vi "俄罗斯方块.vi"() -> ()   [LabVIEW 2021]
uses:
  <vilib>/Utility/config.llb/Read Key (U32).vi
  <vilib>/Utility/config.llb/Read Key (Boolean).vi
  <vilib>/Utility/config.llb/Read Key (I32).vi
  <vilib>/Utility/config.llb/Write Key (U32).vi
  <vilib>/Utility/config.llb/Write Key (Boolean).vi
  <vilib>/Utility/config.llb/Write Key (I32).vi
  <vilib>/Utility/config.llb/NI_LVConfig.lvlib
panel:
  out "扫描代码":i16
  out "键按下状态":bool=TRUE
  out "初始化状态":bool=TRUE
  out "配置文件路径":path
  out "结束状态":bool=TRUE
  out "落下状态":bool=TRUE
  in  "下落触发源":bool=TRUE
  out "速度":i32
  in  "开始/暂停":bool
  out "最多行数":u32
  out "最高分数":u32
  out "行数":u32
  out "分数":u32
  in  "退出":bool
  out "当前形状数组":u32[][](array[colorbox])
  out "Y":i8
  out "X":i8
  out "颜色盒":u32(colorbox)
  in  "新形状触发源":bool=TRUE
  in  "绘图触发源":bool=TRUE
  out "新形状数组":u32[][](array[colorbox])
  out "主窗数组":u32[][](array[colorbox])
  out "二维图片":picture
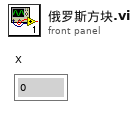
[diagram p1: front panel]
types:
  T1 = typedef "NI_LVConfig.lvlib/Config Data RefNum.ctl" = refnum<k1>
  T2 = enum16{"Left Button", "Center Button", "Right Button", "Window Close"}
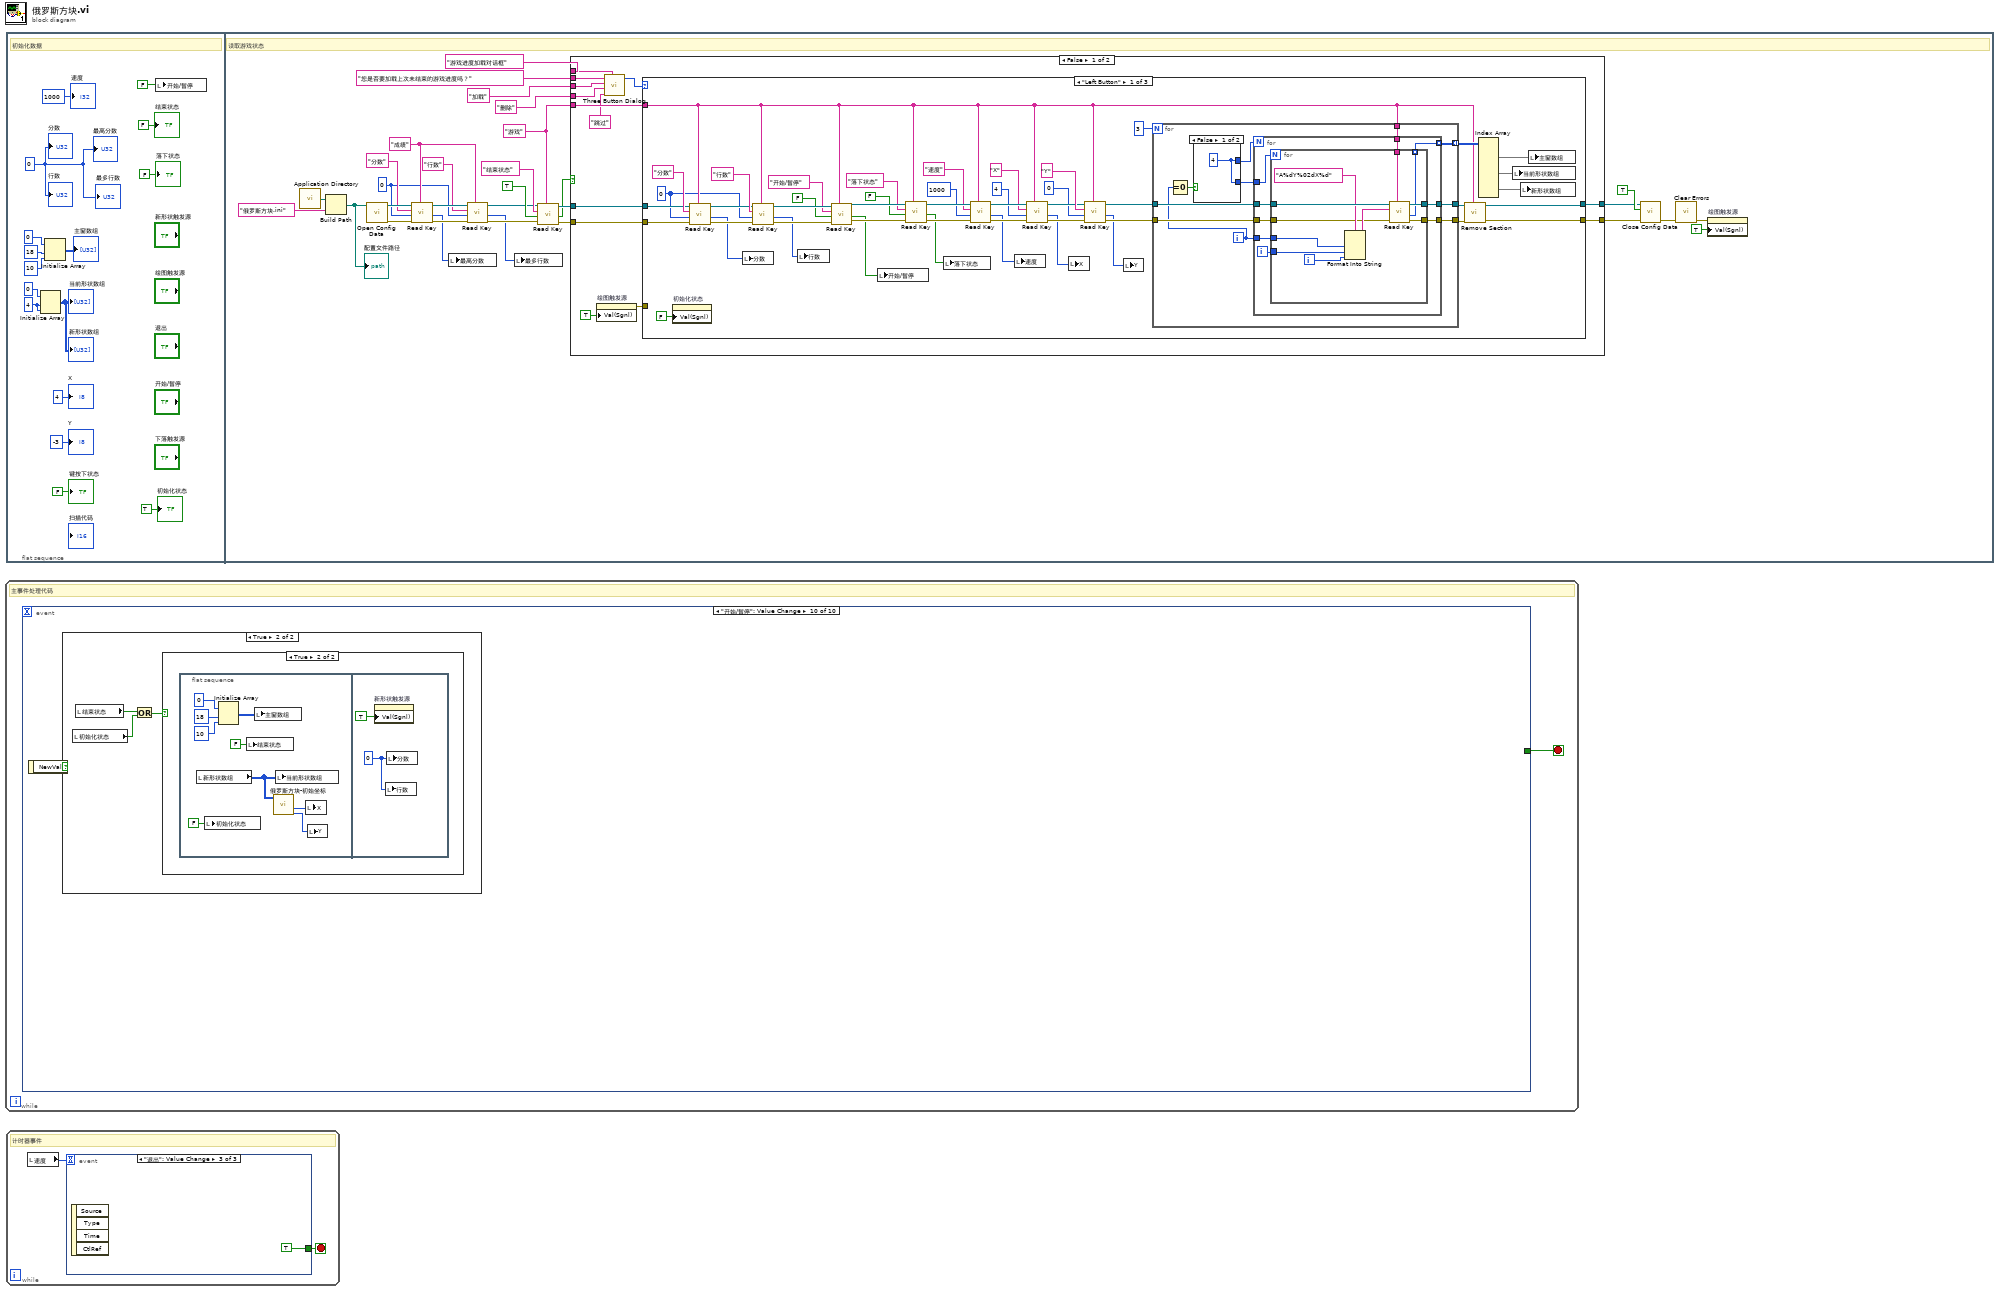
[diagram p0: block diagram]
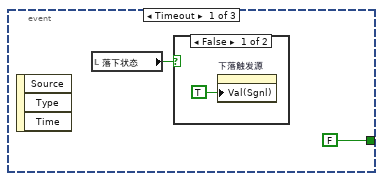
[diagram p2: hidden frame]
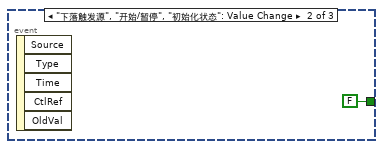
[diagram p4: hidden frame]
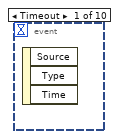
[diagram p5: hidden frame]
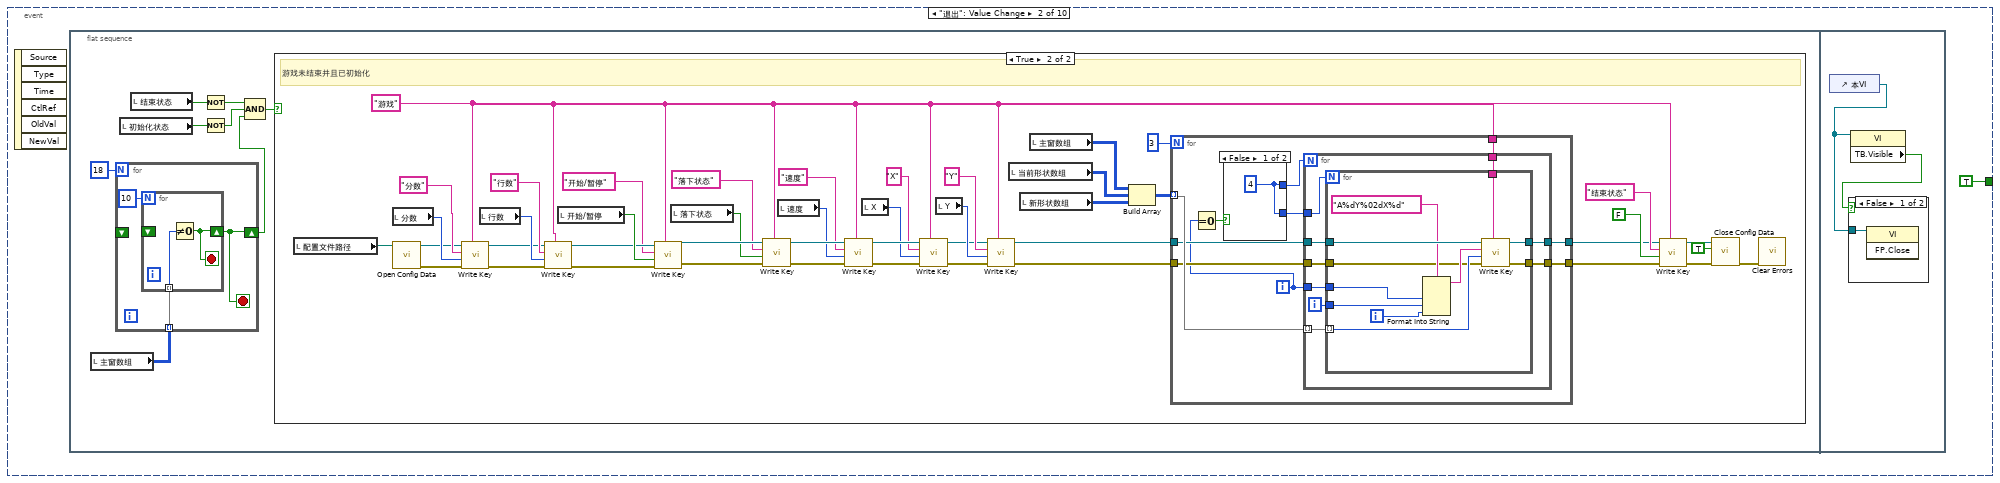
[diagram p6: hidden frame]
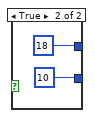
[diagram p8: hidden frame]
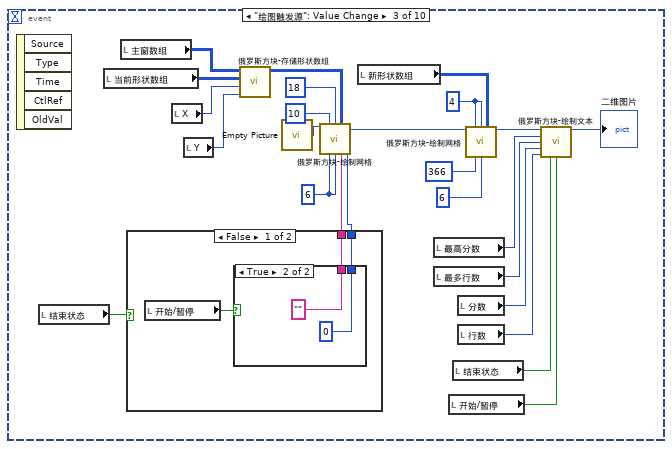
[diagram p10: hidden frame]
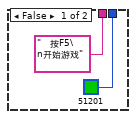
[diagram p11: hidden frame]
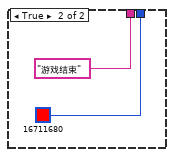
[diagram p12: hidden frame]
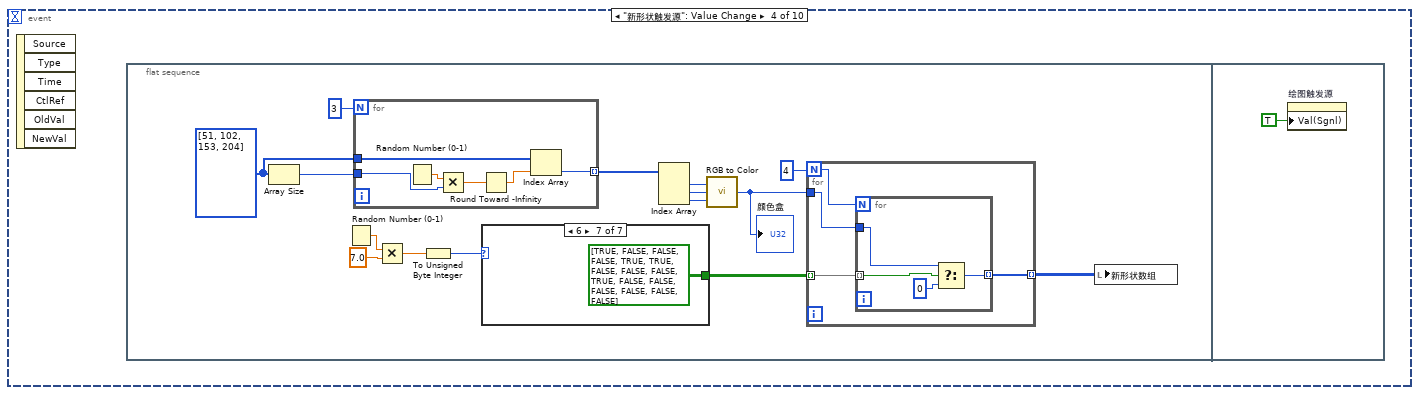
[diagram p13: hidden frame]
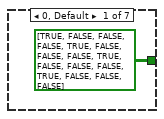
[diagram p14: hidden frame]
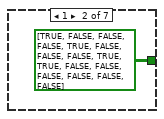
[diagram p15: hidden frame]
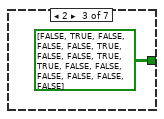
[diagram p16: hidden frame]
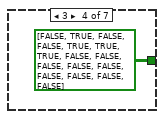
[diagram p17: hidden frame]
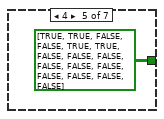
[diagram p18: hidden frame]
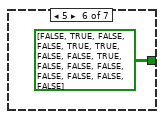
[diagram p19: hidden frame]
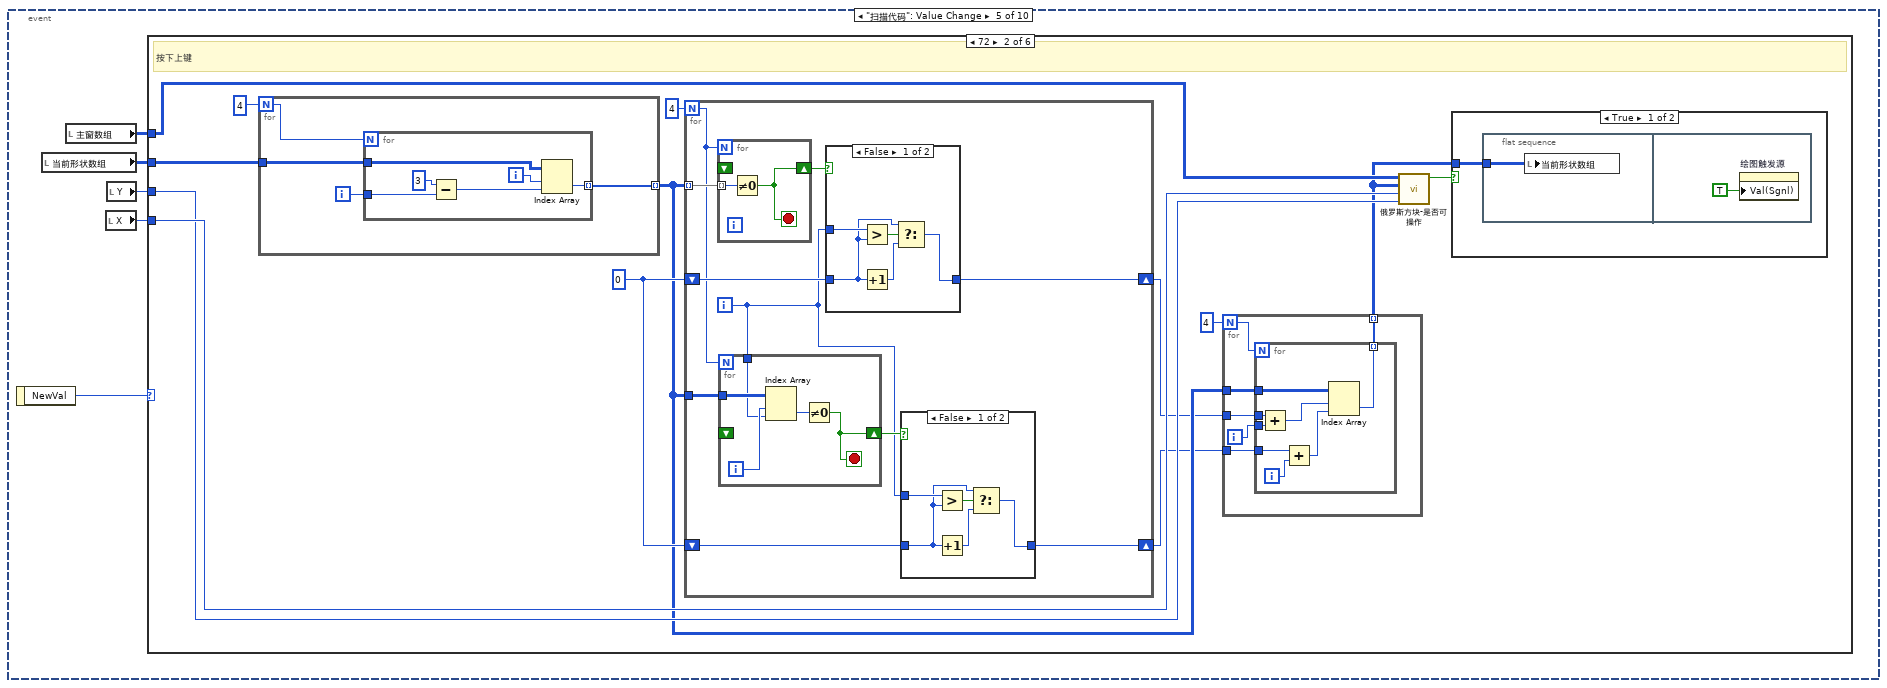
[diagram p20: hidden frame]
diagram:
  n1 = while {
    stop <- w1 stop-if-true
    # "主事件处理代码"
    n2 = event shown="[9] \"开始/暂停\": Value Change" {
      selector: _ -> [_ _ _ _ _ _ _ _ _ _]
      dyn-events: _ -> [_ _ _ _ _ _ _ _ _ _]
      timeout: _ -> [_ _ _ _ _ _ _ _ _ _]
      tunnel: [_ TRUE _ _ _ _ _ _ _ _] -> w1
      event Timeout {
        n3 = event-data() -> ()  [unwired: 1 in, 3 out]
      }
      event "退出": Value Change {
        n4 = event-data() -> ()  [unwired: 1 in, 6 out]
        n5 = flat-sequence {
          frame #0 {
            n6 = local read "主窗数组"() -> (w4:u32[][])
            n7 = for {
              N: 18 -> [_]
              shift-right: [w11] -> w3
              shift-left: _ -> [_]
              tunnel: w4 -> [w12] mode=indexing
              stop <- w11 stop-if-true
              n8 = for {
                N: 10 -> [_]
                shift-right: [w14] -> w11
                shift-left: _ -> [_]
                tunnel: w12 -> [w15] mode=indexing
                stop <- w14 stop-if-true
                n9 = Not Equal To 0?(x=w15) -> (x != 0?=w14:bool)
              }
            }
            n10 = local read "初始化状态"() -> (w7:bool)
            n11 = local read "结束状态"() -> (w8:bool)
            n12 = Not(x=w8) -> (.not. x?=w9:bool)
            n13 = Not(x=w7) -> (.not. x?=w6:bool)
            n14 = Compound Arithmetic op=AND ("复合运算")(w9, w6, w3) -> (w10:bool)
            n15 = case shown="True" w10 {
              frame False {
                # "不保存状态"
              }
              frame True {
                w16 = "游戏" ("section")
                # "游戏未结束并且已初始化"
                n16 = local read "配置文件路径"() -> (w60:path)
                n17 = local read "分数"() -> (w57:u32)
                n18 = call <vilib>:"Open Config Data.vi"("configuration file path"=w60) -> ("error out"=w46:errorcluster, "refnum"=w47:T1)  [unwired: 8 in, 1 out]
                n19 = call-poly <vilib>:"Write Key.vi"("section"=w16, "error in (no error)"=w46, "value"=w57, "key"="分数", "refnum"=w47) -> ("error out"=w53:errorcluster, "refnum out"=w54:T1)  [unwired: 4 in, 1 out]
                n20 = local read "行数"() -> (w56:u32)
                n21 = call-poly <vilib>:"Write Key.vi"("section"=w16, "error in (no error)"=w53, "value"=w56, "key"="行数", "refnum"=w54) -> ("error out"=w44:errorcluster, "refnum out"=w43:T1)  [unwired: 4 in, 1 out]
                n22 = local read "开始/暂停"() -> (w45:bool)
                n23 = call-poly <vilib>:"Write Key.vi"("section"=w16, "error in (no error)"=w44, "value"=w45, "key"="开始/暂停", "refnum"=w43) -> ("error out"=w40:errorcluster, "refnum out"=w41:T1)  [unwired: 4 in, 1 out]
                n24 = local read "落下状态"() -> (w39:bool)
                n25 = call-poly <vilib>:"Write Key.vi"("section"=w16, "error in (no error)"=w40, "value"=w39, "key"="落下状态", "refnum"=w41) -> ("error out"=w36:errorcluster, "refnum out"=w37:T1)  [unwired: 4 in, 1 out]
                n26 = local read "速度"() -> (w34:i32)
                n27 = call-poly <vilib>:"Write Key.vi"("section"=w16, "error in (no error)"=w36, "value"=w34, "key"="速度", "refnum"=w37) -> ("error out"=w33:errorcluster, "refnum out"=w32:T1)  [unwired: 4 in, 1 out]
                n28 = local read "X"() -> (w30:i8)
                n29 = call-poly <vilib>:"Write Key.vi"("section"=w16, "error in (no error)"=w33, "value"=w30, "key"="X", "refnum"=w32) -> ("error out"=w29:errorcluster, "refnum out"=w26:T1)  [unwired: 4 in, 1 out]
                n30 = local read "Y"() -> (w28:i8)
                n31 = call-poly <vilib>:"Write Key.vi"("section"=w16, "error in (no error)"=w29, "value"=w28, "key"="Y", "refnum"=w26) -> ("error out"=w19:errorcluster, "refnum out"=w20:T1)  [unwired: 4 in, 1 out]
                n32 = local read "当前形状数组"() -> (w24:u32[][])
                n33 = local read "新形状数组"() -> (w25:u32[][])
                n34 = local read "主窗数组"() -> (w23:u32[][])
                n35 = Build Array(w23, w24, w25) -> (w22:u32[][][])
                n36 = for {
                  N: 3 -> [_]
                  tunnel: w22 -> [w70] mode=indexing
                  tunnel: w20 -> [w69]
                  tunnel: w19 -> [w68]
                  tunnel: [w67] -> w18
                  tunnel: [w66] -> w17
                  tunnel: w16 -> [w65]
                  i -> [w64]
                  n37 = Equal To 0?(x=w64) -> (x = 0?=w63:bool)
                  n38 = case shown="False" w63 {
                    tunnel: [w71 18] -> w62
                    tunnel: [w71 10] -> w61
                    frame False {
                      w71 = 4
                    }
                    frame True {
                    }
                  }
                  n39 = for {
                    N: w62 -> [_]
                    tunnel: w61 -> [w82]
                    tunnel: w70 -> [w81] mode=indexing
                    tunnel: w69 -> [w80]
                    tunnel: w64 -> [w78]
                    tunnel: w68 -> [w77]
                    tunnel: [w76] -> w67
                    tunnel: [w75] -> w66
                    tunnel: w65 -> [w74]
                    i -> [w79]
                    n40 = for {
                      N: w82 -> [_]
                      tunnel: w81 -> [w87] mode=indexing
                      tunnel: w80 -> [w93]
                      tunnel: w79 -> [w91]
                      tunnel: w78 -> [w90]
                      tunnel: w77 -> [w86]
                      tunnel: [w85] -> w76
                      tunnel: [w84] -> w75
                      tunnel: w74 -> [w83]
                      i -> [w89]
                      n41 = Format Into String(format string="A%dY%02dX%d" ("格式字符串"), w90, w91, w89) -> (resulting string=w92:string)  [unwired: 2 in, 1 out]
                      n42 = call-poly <vilib>:"Write Key.vi"("section"=w83, "error in (no error)"=w86, "value"=w87, "key"=w92, "refnum"=w93) -> ("error out"=w84:errorcluster, "refnum out"=w85:T1)  [unwired: 4 in, 1 out]
                    }
                  }
                }
                n43 = call-poly <vilib>:"Write Key.vi"("section"=w16, "error in (no error)"=w17, "value"=FALSE, "key"="结束状态", "refnum"=w18) -> ("error out"=w52:errorcluster, "refnum out"=w51:T1)  [unwired: 4 in, 1 out]
                n44 = call <vilib>:"Close Config Data.vi"("error in (no error)"=w52, "write file if changed (T)"=TRUE, "refnum"=w51) -> ("error out"=w59:errorcluster)  [unwired: 7 in, 1 out]
                n45 = call <vilib>:"Clear Errors.vi"("error in (no error)"=w59) -> ()  [unwired: 5 in, 2 out]
              }
            }
          }
          frame #1 {
            n46 = control-ref of="本VI"() -> (w95:refnum<vi>)
            n47 = property class="VI"(reference=w95) -> ("TB.Visible"=w94:bool)  [unwired: 1 in, 2 out]
            n48 = case shown="False" w94 {
              tunnel: w95 -> [w96 _]
              frame False {
                n49 = invoke class="VI" method="FP.Close"(reference=w96) -> ()  [unwired: 2 in, 3 out]
              }
              frame True {
              }
            }
          }
        }
      }
      event "绘图触发源": Value Change {
        w114 = i16 4 ("yN")
        w108 = i16 6 ("xOffset")
        n50 = event-data() -> ()  [unwired: 1 in, 5 out]
        n51 = local read "结束状态"() -> (w111:bool)
        n52 = local read "当前形状数组"() -> (w97:u32[][])
        n53 = local read "主窗数组"() -> (w98:u32[][])
        n54 = case shown="False" w111 {
          tunnel: [w124 "游戏结束"] -> w110
          tunnel: [w123 u32 16711680 ("消息颜色")] -> w109
          frame False {
            n55 = local read "开始/暂停"() -> (w122:bool)
            n56 = case shown="True" w122 {
              tunnel: ["　按F5\n开始游戏" ""] -> w124
              tunnel: [u32 51201 ("消息颜色") u32 0 ("消息颜色")] -> w123
              frame False {
              }
              frame True {
              }
            }
          }
          frame True {
          }
        }
        n57 = local read "X"() -> (w117:i8)
        n58 = local read "Y"() -> (w116:i8)
        n59 = call "俄罗斯方块-存储形状数组.vi"("Y"=w116, "X"=w117, "当前形状数组"=w97, "主窗数组输入"=w98) -> ("主窗数组输出"=w99:u32[][])  [unwired: 4 in, 1 out]
        n60 = call "Empty Picture"() -> ("empty picture"=w120:picture)
        n61 = call "俄罗斯方块-绘制网格.vi"("图片输入"=w120, "xN"=i16 10, "yN"=i16 18, "数组"=w99, "xOffset"=w108, "yOffset"=w108, "消息文本"=w110, "消息颜色"=w109) -> ("图片输出"=w121:picture)  [unwired: 7 in]
        n62 = local read "新形状数组"() -> (w113:u32[][])
        n63 = local read "最高分数"() -> (w102:u32)
        n64 = local read "最多行数"() -> (w103:u32)
        n65 = local read "开始/暂停"() -> (w100:bool)
        n66 = local read "结束状态"() -> (w101:bool)
        n67 = local read "分数"() -> (w104:u32)
        n68 = local read "行数"() -> (w105:u32)
        n69 = call "俄罗斯方块-绘制网格.vi"("图片输入"=w121, "xN"=w114, "yN"=w114, "数组"=w113, "xOffset"=i16 366, "yOffset"=i16 6) -> ("图片输出"=w107:picture)  [unwired: 9 in]
        n70 = call "俄罗斯方块-绘制文本.vi"("输入图片"=w107, "最高分数"=w102, "最多行数"=w103, "分数"=w104, "行数"=w105, "结束状态"=w101, "开始/暂停"=w100) -> ("输出图片"=→"二维图片":picture)  [unwired: 8 in]
      }
      event "新形状触发源": Value Change {
        n71 = event-data() -> ()  [unwired: 1 in, 6 out]
        n72 = flat-sequence {
          frame #0 {
            w133 = u8[] [51, 102, 153, 204]
            n73 = Array Size(array=w133) -> (size(s)=w134:i32)
            n74 = Random Number (0-1)() -> (number: 0 to 1=w139:dbl)
            n75 = for {
              N: 3 -> [_]
              tunnel: [w163] -> w144 mode=indexing
              tunnel: w134 -> [w165]
              tunnel: w133 -> [w164]
              n76 = Random Number (0-1)() -> (number: 0 to 1=w166:dbl)
              n77 = Multiply(x=w166, y=w165) -> (x*y=w161:dbl)
              n78 = Round Toward -Infinity(1:w161) -> (0:w162:dbl)
              n79 = Index Array(array=w164, index=w162) -> (element=w163:u8)
            }
            n80 = Multiply(x=w139, y=7.0) -> (x*y=w138:dbl)
            n81 = To Unsigned Byte Integer(number=w138) -> (unsigned 8bit integer=w140:u8)
            n82 = case shown="6" w140 {
              tunnel: [bool[][] [[TRUE, FALSE, FALSE, FALSE], [TRUE, FALSE, FALSE, FALSE], [TRUE, FALSE, FALSE, FALSE], [TRUE, FALSE, FALSE, FALSE]] bool[][] [[TRUE, FALSE, FALSE, FALSE], [TRUE, FALSE, FALSE, FALSE], [TRUE, TRUE, FALSE, FALSE], [FALSE, FALSE, FALSE, FALSE]] bool[][] [[FALSE, TRUE, FALSE, FALSE], [FALSE, TRUE, FALSE, FALSE], [TRUE, TRUE, FALSE, FALSE], [FALSE, FALSE, FALSE, FALSE]] bool[][] [[FALSE, TRUE, FALSE, FALSE], [TRUE, TRUE, TRUE, FALSE], [FALSE, FALSE, FALSE, FALSE], [FALSE, FALSE, FALSE, FALSE]] bool[][] [[TRUE, TRUE, FALSE, FALSE], [TRUE, TRUE, FALSE, FALSE], [FALSE, FALSE, FALSE, FALSE], [FALSE, FALSE, FALSE, FALSE]] bool[][] [[FALSE, TRUE, FALSE, FALSE], [TRUE, TRUE, FALSE, FALSE], [TRUE, FALSE, FALSE, FALSE], [FALSE, FALSE, FALSE, FALSE]] bool[][] [[TRUE, FALSE, FALSE, FALSE], [TRUE, TRUE, FALSE, FALSE], [FALSE, TRUE, FALSE, FALSE], [FALSE, FALSE, FALSE, FALSE]]] -> w135
              frame 0, Default {
              }
              frame 1 {
              }
              frame 2 {
              }
              frame 3 {
              }
              frame 4 {
              }
              frame 5 {
              }
              frame 6 {
              }
            }
            n83 = Index Array(array=w144) -> (element #1=w143:u8, element #2=w142:u8, element #3=w141:u8)  [unwired: 3 in]
            n84 = call <vilib>:"RGB to Color.vi"("B"=w141, "G"=w142, "R"=w143) -> ("Color"=w132:u32)
            "颜色盒" <- w132
            n85 = for {
              N: 4 -> [w146]
              tunnel: w132 -> [w149]
              tunnel: w135 -> [w148] mode=indexing
              tunnel: [w147] -> w131 mode=indexing
              n86 = for {
                N: w146 -> [_]
                tunnel: w149 -> [w153]
                tunnel: w148 -> [w151] mode=indexing
                tunnel: [w150] -> w147 mode=indexing
                n87 = Select(t=w153, s=w151, f=u32 0) -> (s? t:f=w150:u32)
              }
            }
            n88 = local write "新形状数组"(w131) -> ()
          }
          frame #1 {
            n89 = property on="绘图触发源" class="Bool (strict)"("Val(Sgnl)"=TRUE ("绘图触发源")) -> ()  [unwired: 2 in, 2 out]
          }
        }
      }
      event "扫描代码": Value Change {
        n90 = event-data() -> ("NewVal"=w172:i16)  [unwired: 1 in]
        n91 = local read "当前形状数组"() -> (w170:u32[][])
        n92 = local read "主窗数组"() -> (w171:u32[][])
        n93 = local read "X"() -> (w169:i8)
        n94 = local read "Y"() -> (w168:i8)
        n95 = case shown="72" w172 {
          tunnel: w171 -> [_ w185 _ _ w249 w258]
          tunnel: w170 -> [_ w180 _ _ w248 w257]
          tunnel: w169 -> [_ w184 _ _ w246 w255]
          tunnel: w168 -> [_ w183 _ _ w247 w256]
          frame 0, Default {
          }
          frame 72 {
            w178 = 0
            # "按下上键"
            n96 = for {
              N: 4 -> [w231]
              tunnel: [w232] -> w177 mode=indexing
              tunnel: w180 -> [w230]
              i -> [w229]
              n97 = for {
                N: w231 -> [_]
                tunnel: [w238] -> w232 mode=indexing
                tunnel: w230 -> [w237]
                tunnel: w229 -> [w233]
                i -> [w234]
                n98 = Subtract(x=i8 3, y=w233) -> (x-y=w235:i32)
                n99 = Index Array(array=w237, index (row)=w234, index (col)=w235) -> (element=w238:u32)
              }
            }
            n100 = for {
              N: 4 -> [w205]
              tunnel: w177 -> [w209] mode=indexing
              shift-right: [w206] -> w175
              shift-left: w178 -> [w207]
              tunnel: w177 -> [w204]
              shift-right: [w202] -> w174
              shift-left: w178 -> [w201]
              i -> [w200]
              n101 = for {
                N: w205 -> [_]
                tunnel: w209 -> [w228] mode=indexing
                shift-right: [w227] -> w208
                shift-left: _ -> [_]
                stop <- w227 stop-if-true
                n102 = Not Equal To 0?(x=w228) -> (x != 0?=w227:bool)
              }
              n103 = for {
                N: w205 -> [_]
                tunnel: w204 -> [w220]
                tunnel: w200 -> [w218]
                shift-right: [w216] -> w203
                shift-left: _ -> [_]
                i -> [w219]
                stop <- w216 stop-if-true
                n104 = Index Array(array=w220, index (row)=w219, index (col)=w218) -> (element=w217:u32)
                n105 = Not Equal To 0?(x=w217) -> (x != 0?=w216:bool)
              }
              n106 = case shown="False" w208 {
                tunnel: w207 -> [w223 w226]
                tunnel: [w221 w226] -> w206
                tunnel: w200 -> [w224 _]
                frame False {
                  n107 = Greater?(x=w224, y=w223) -> (0:w225:bool)
                  n108 = Increment(x=w223) -> (x+1=w222:i32)
                  n109 = Select(t=w223, s=w225, f=w222) -> (s? t:f=w221:i32)
                }
                frame True {
                }
              }
              n110 = case shown="False" w203 {
                tunnel: w201 -> [w212 w215]
                tunnel: [w210 w215] -> w202
                tunnel: w200 -> [w213 _]
                frame False {
                  n111 = Greater?(x=w213, y=w212) -> (0:w214:bool)
                  n112 = Increment(x=w212) -> (x+1=w211:i32)
                  n113 = Select(t=w212, s=w214, f=w211) -> (s? t:f=w210:i32)
                }
                frame True {
                }
              }
            }
            n114 = for {
              N: 4 -> [w190]
              tunnel: w177 -> [w191]
              tunnel: w175 -> [w188]
              tunnel: w174 -> [w187]
              tunnel: [w186] -> w173 mode=indexing
              i -> [w189]
              n115 = for {
                N: w190 -> [_]
                tunnel: w191 -> [w199]
                tunnel: w189 -> [w197]
                tunnel: w188 -> [w196]
                tunnel: w187 -> [w194]
                tunnel: [w192] -> w186 mode=indexing
                i -> [w195]
                n116 = Add(x=w196, y=w197) -> (x+y=w198:i32)
                n117 = Add(x=w194, y=w195) -> (x+y=w193:i32)
                n118 = Index Array(array=w199, index (row)=w198, index (col)=w193) -> (element=w192:u32)
              }
            }
            n119 = call "俄罗斯方块-是否可操作.vi"("Y"=w183, "X"=w184, "形状数组"=w173, "主窗数组"=w185) -> ("是否可操作"=w182:bool)  [unwired: 7 in]
            n120 = case shown="True" w182 {
              tunnel: w173 -> [w239 _]
              frame True {
                n121 = flat-sequence {
                  tunnel: w239 -> [w240]
                  frame #0 {
                    n122 = local write "当前形状数组"(w240) -> ()
                  }
                  frame #1 {
                    n123 = property on="绘图触发源" class="Bool (strict)"("Val(Sgnl)"=TRUE ("值(信号)")) -> ()  [unwired: 2 in, 2 out]
                  }
                }
              }
              frame False {
              }
            }
          }
          frame 57 {
            # "空格键"
            n124 = flat-sequence {
              frame #0 {
                n125 = local write "落下状态"(TRUE ("落下状态")) -> ()
              }
              frame #1 {
                n126 = property on="下落触发源" class="Bool (strict)"("Val(Sgnl)"=TRUE ("值(信号)")) -> ()  [unwired: 2 in, 2 out]
              }
            }
          }
          frame 80 {
            # "按下下键"
            n127 = property on="下落触发源" class="Bool (strict)"("Val(Sgnl)"=TRUE ("值(信号)")) -> ()  [unwired: 2 in, 2 out]
          }
          frame 75 {
            # "按下左键"
            n128 = Decrement(x=w246) -> (x-1=w245:i8)
            n129 = call "俄罗斯方块-是否可操作.vi"("Y"=w247, "X"=w245, "形状数组"=w248, "主窗数组"=w249) -> ("是否可操作"=w250:bool)  [unwired: 7 in]
            n130 = case shown="True" w250 {
              tunnel: w245 -> [_ w251]
              frame False {
              }
              frame True {
                n131 = flat-sequence {
                  tunnel: w251 -> [w252]
                  frame #0 {
                    n132 = local write "X"(w252) -> ()
                  }
                  frame #1 {
                    n133 = property on="绘图触发源" class="Bool (strict)"("Val(Sgnl)"=TRUE ("值(信号)")) -> ()  [unwired: 2 in, 2 out]
                  }
                }
              }
            }
          }
          frame 77 {
            # "按下右键"
            n134 = Increment(x=w255) -> (x+1=w254:i8)
            n135 = call "俄罗斯方块-是否可操作.vi"("Y"=w256, "X"=w254, "形状数组"=w257, "主窗数组"=w258) -> ("是否可操作"=w259:bool)  [unwired: 7 in]
            n136 = case shown="True" w259 {
              tunnel: w254 -> [_ w260]
              frame False {
              }
              frame True {
                n137 = flat-sequence {
                  tunnel: w260 -> [w261]
                  frame #0 {
                    n138 = local write "X"(w261) -> ()
                  }
                  frame #1 {
                    n139 = property on="绘图触发源" class="Bool (strict)"("Val(Sgnl)"=TRUE ("值(信号)")) -> ()  [unwired: 2 in, 2 out]
                  }
                }
              }
            }
          }
        }
      }
      event Key Down {
        n140 = event-data() -> ("ScanCode"=w263:i16)  [unwired: 1 in]
        n141 = case shown="63" w263 {
          selector: w263 -> [w264 _ _]
          frame 0, Default {
            n142 = local read "开始/暂停"() -> (w268:bool)
            n143 = local read "落下状态"() -> (w266:bool)
            n144 = Not(x=w266) -> (.not. x?=w267:bool)
            n145 = And(x=w268, y=w267) -> (x .and. y?=w265:bool)
            n146 = case shown="True" w265 {
              tunnel: w264 -> [_ w269]
              frame False {
              }
              frame True {
                n147 = property on="扫描代码" class="DigNum (strict)"("Val(Sgnl)"=w269) -> ()  [unwired: 2 in, 2 out]
              }
            }
            n148 = local write "键按下状态"(w265) -> ()
          }
          frame 63 {
            # "按下F5键"
            n149 = local read "开始/暂停"() -> (w270:bool)
            n150 = Not(x=w270) -> (.not. x?=w271:bool)
            n151 = property on="开始/暂停" class="Bool (strict)"("Val(Sgnl)"=w271) -> ()  [unwired: 2 in, 2 out]
          }
          frame 62 {
            # "按下F4键"
            n152 = property on="退出" class="Bool (strict)"("Val(Sgnl)"=TRUE ("值(信号)")) -> ()  [unwired: 2 in, 2 out]
          }
        }
      }
      event event type 5.0.x8000000b {
        n153 = event-data() -> ("ScanCode"=w275:i16)  [unwired: 1 in]
        n154 = local read "落下状态"() -> (w277:bool)
        n155 = local read "键按下状态"() -> (w276:bool)
        n156 = local read "开始/暂停"() -> (w279:bool)
        n157 = Not(x=w277) -> (.not. x?=w278:bool)
        n158 = Compound Arithmetic op=AND ("复合运算")(w279, w278, w276) -> (w274:bool)
        n159 = case shown="True" w274 {
          tunnel: w275 -> [_ w280]
          frame False {
          }
          frame True {
            n160 = property on="扫描代码" class="DigNum (strict)"("Val(Sgnl)"=w280) -> ()  [unwired: 2 in, 2 out]
          }
        }
        n161 = Not(x=w274) -> (.not. x?=w273:bool)
        n162 = event-data("Discard?"=w273) -> ()  [unwired: 1 in, 1 out]
      }
      event Key Up {
        n163 = event-data() -> ()  [unwired: 1 in, 1 out]
        n164 = local write "键按下状态"(FALSE ("键按下状态")) -> ()
      }
      event "下落触发源": Value Change {
        n165 = event-data() -> ()  [unwired: 1 in, 3 out]
        n166 = local read "开始/暂停"() -> (w282:bool)
        n167 = case shown="True" w282 {
          frame False {
          }
          frame True {
            n168 = local read "当前形状数组"() -> (w287:u32[][])
            n169 = local read "主窗数组"() -> (w288:u32[][])
            n170 = local read "Y"() -> (w285:i8)
            n171 = local read "X"() -> (w286:i8)
            n172 = Increment(x=w285) -> (x+1=w283:i8)
            n173 = call "俄罗斯方块-是否可操作.vi"("Y"=w283, "X"=w286, "形状数组"=w287, "主窗数组"=w288) -> ("是否可操作"=w284:bool)  [unwired: 7 in]
            n174 = case shown="True" w284 {
              tunnel: w283 -> [_ w359]
              tunnel: w285 -> [w289 _]
              frame False {
                # "不可下落，存储，如果结束把结束状态设置为F，否则创建新形状并重新下落"
                n175 = stacked-sequence {
                  tunnel: w289 -> [w296 _ _]
                  frame #0 {
                    # "存储并消除满行和记分"
                    n176 = local read "当前形状数组"() -> (w299:u32[][])
                    n177 = local read "主窗数组"() -> (w298:u32[][])
                    n178 = local read "X"() -> (w297:i8)
                    n179 = call "俄罗斯方块-存储形状数组.vi"("Y"=w296, "X"=w297, "当前形状数组"=w299, "主窗数组输入"=w298) -> ("是否溢出"=w290:bool, "主窗数组输出"=w295:u32[][])  [unwired: 4 in]
                    n180 = local write "结束状态"(w290) -> ()
                    n181 = call "俄罗斯方块-消除满行.vi"("输入数组"=w295) -> ("行数"=w291:u32, "分数"=w292:u32, "输出数组"=w294:u32[][])  [unwired: 8 in]
                    n182 = Greater Than 0?(x=w291) -> (x > 0?=w293:bool)
                    n183 = local write "主窗数组"(w294) -> ()
                    n184 = case shown="True" w293 {
                      tunnel: w292 -> [_ w314]
                      tunnel: w291 -> [_ w315]
                      frame False {
                      }
                      frame True {
                        w308 = 50.0 ("y")
                        n185 = local read "分数"() -> (w305:u32)
                        n186 = local read "行数"() -> (w304:u32)
                        n187 = local read "最多行数"() -> (w302:u32)
                        n188 = local read "最高分数"() -> (w303:u32)
                        n189 = Add(x=w314, y=w305) -> (x+y=w301:u32)
                        n190 = Add(x=w304, y=w315) -> (x+y=w300:u32)
                        n191 = Subtract(x=1000.0, y=w300) -> (x-y=w306:dbl)
                        n192 = Greater?(x=w306, y=w308) -> (0:w310:bool)
                        n193 = Greater?(x=w301, y=w303) -> (0:w312:bool)
                        n194 = Select(t=w306, s=w310, f=w308) -> (s? t:f=w307:dbl)
                        n195 = Greater?(x=w300, y=w302) -> (0:w311:bool)
                        n196 = local write "行数"(w300) -> ()
                        n197 = local write "速度"(w307) -> ()
                        n198 = Or(x=w312, y=w311) -> (x .or. y?=w313:bool)
                        n199 = case shown="True" w313 {
                          tunnel: w312 -> [_ w338]
                          tunnel: w301 -> [_ w337]
                          tunnel: w303 -> [_ w336]
                          tunnel: w311 -> [_ w335]
                          tunnel: w300 -> [_ w334]
                          tunnel: w302 -> [_ w333]
                          frame False {
                          }
                          frame True {
                            w326 = "成绩" ("section")
                            n200 = Select(t=w337, s=w338, f=w336) -> (s? t:f=w317:u32)
                            n201 = Select(t=w334, s=w335, f=w333) -> (s? t:f=w316:u32)
                            n202 = local read "配置文件路径"() -> (w332:path)
                            n203 = local write "最多行数"(w316) -> ()
                            n204 = local write "最高分数"(w317) -> ()
                            n205 = call <vilib>:"Open Config Data.vi"("configuration file path"=w332) -> ("error out"=w327:errorcluster, "refnum"=w328:T1)  [unwired: 8 in, 1 out]
                            n206 = call-poly <vilib>:"Write Key.vi"("section"=w326, "error in (no error)"=w327, "value"=w316, "key"="行数", "refnum"=w328) -> ("error out"=w329:errorcluster, "refnum out"=w330:T1)  [unwired: 4 in, 1 out]
                            n207 = call-poly <vilib>:"Write Key.vi"("section"=w326, "error in (no error)"=w329, "value"=w317, "key"="分数", "refnum"=w330) -> ("error out"=w321:errorcluster, "refnum out"=w322:T1)  [unwired: 4 in, 1 out]
                            n208 = call <vilib>:"Remove Section.vi"("section"="游戏", "error in (no error)"=w321, "refnum"=w322) -> ("error out"=w318:errorcluster, "refnum out"=w319:T1)  [unwired: 6 in, 1 out]
                            n209 = call <vilib>:"Close Config Data.vi"("error in (no error)"=w318, "write file if changed (T)"=TRUE, "refnum"=w319) -> ("error out"=w331:errorcluster)  [unwired: 7 in, 1 out]
                            n210 = call <vilib>:"Clear Errors.vi"("error in (no error)"=w331) -> ()  [unwired: 5 in, 2 out]
                          }
                        }
                        n211 = local write "分数"(w301) -> ()
                      }
                    }
                  }
                  frame #1 {
                    # "初始化落下状态、XY坐标、把新形状作为当前形状"
                    n212 = local read "结束状态"() -> (w339:bool)
                    n213 = local write "落下状态"(FALSE ("落下状态")) -> ()
                    n214 = case shown="False" w339 {
                      frame False {
                        n215 = local read "新形状数组"() -> (w343:u32[][])
                        n216 = call "俄罗斯方块-初始坐标.vi"("输入形状数组"=w343) -> ("Y"=w341:i8, "X"=w342:i8)  [unwired: 9 in]
                        n217 = local write "当前形状数组"(w343) -> ()
                        n218 = local write "X"(w342) -> ()
                        n219 = local write "Y"(w341) -> ()
                      }
                      frame True {
                      }
                    }
                  }
                  frame #2 {
                    # "判断游戏是否结束"
                    n220 = local read "当前形状数组"() -> (w350:u32[][])
                    n221 = local read "主窗数组"() -> (w351:u32[][])
                    n222 = local read "X"() -> (w349:i8)
                    n223 = local read "Y"() -> (w348:i8)
                    n224 = call "俄罗斯方块-是否可操作.vi"("Y"=w348, "X"=w349, "形状数组"=w350, "主窗数组"=w351) -> ("是否可操作"=w345:bool)  [unwired: 7 in]
                    n225 = local read "结束状态"() -> (w347:bool)
                    n226 = Not(x=w347) -> (.not. x?=w346:bool)
                    n227 = And(x=w345, y=w346) -> (x .and. y?=w344:bool)
                    n228 = case shown="False" w344 {
                      frame False {
                        # "游戏结束"
                        n229 = flat-sequence {
                          frame #0 {
                            w355 = 4 ("维数大小")
                            n230 = Initialize Array(u32 0 ("元素"), w355, w355) -> (w353:u32[][])
                            n231 = local write "开始/暂停"(FALSE ("开始/暂停")) -> ()
                            n232 = local write "结束状态"(TRUE ("结束状态")) -> ()
                            n233 = local write "当前形状数组"(w353) -> ()
                          }
                          frame #1 {
                            n234 = property on="绘图触发源" class="Bool (strict)"("Val(Sgnl)"=TRUE ("值(信号)")) -> ()  [unwired: 2 in, 2 out]
                          }
                        }
                      }
                      frame True {
                        # "未结束，产生新形状数据"
                        n235 = property on="新形状触发源" class="Bool (strict)"("Val(Sgnl)"=TRUE ("值(信号)")) -> ()  [unwired: 2 in, 2 out]
                      }
                    }
                  }
                }
              }
              frame True {
                n236 = flat-sequence {
                  tunnel: w359 -> [w360]
                  frame #0 {
                    n237 = local write "Y"(w360) -> ()
                  }
                  frame #1 {
                    n238 = local read "落下状态"() -> (w361:bool)
                    n239 = case shown="False" w361 {
                      frame False {
                        n240 = property on="绘图触发源" class="Bool (strict)"("Val(Sgnl)"=FALSE ("值(信号)")) -> ()  [unwired: 2 in, 2 out]
                      }
                      frame True {
                        n241 = property on="下落触发源" class="Bool (strict)"("Val(Sgnl)"=TRUE ("值(信号)")) -> ()  [unwired: 2 in, 2 out]
                      }
                    }
                  }
                }
              }
            }
          }
        }
      }
      event "开始/暂停": Value Change {
        n242 = event-data() -> ("NewVal"=w364:bool)  [unwired: 1 in]
        n243 = case shown="True" w364 {
          frame False {
            n244 = property on="绘图触发源" class="Bool (strict)"("Val(Sgnl)"=FALSE ("值(信号)")) -> ()  [unwired: 2 in, 2 out]
          }
          frame True {
            n245 = local read "初始化状态"() -> (w367:bool)
            n246 = local read "结束状态"() -> (w368:bool)
            n247 = Or(x=w368, y=w367) -> (x .or. y?=w366:bool)
            n248 = case shown="True" w366 {
              frame False {
                n249 = local read "落下状态"() -> (w369:bool)
                n250 = case shown="True" w369 {
                  frame False {
                    n251 = property on="绘图触发源" class="Bool (strict)"("Val(Sgnl)"=FALSE ("值(信号)")) -> ()  [unwired: 2 in, 2 out]
                  }
                  frame True {
                    n252 = property on="下落触发源" class="Bool (strict)"("Val(Sgnl)"=TRUE ("值(信号)")) -> ()  [unwired: 2 in, 2 out]
                  }
                }
              }
              frame True {
                n253 = flat-sequence {
                  frame #0 {
                    n254 = local read "新形状数组"() -> (w375:u32[][])
                    n255 = local write "初始化状态"(FALSE ("初始化状态")) -> ()
                    n256 = Initialize Array(u32 0 ("元素"), 18 ("维数大小"), 10 ("维数大小")) -> (w377:u32[][])
                    n257 = local write "结束状态"(FALSE ("结束状态")) -> ()
                    n258 = local write "主窗数组"(w377) -> ()
                    n259 = call "俄罗斯方块-初始坐标.vi"("输入形状数组"=w375) -> ("Y"=w373:i8, "X"=w374:i8)  [unwired: 9 in]
                    n260 = local write "当前形状数组"(w375) -> ()
                    n261 = local write "X"(w374) -> ()
                    n262 = local write "Y"(w373) -> ()
                  }
                  frame #1 {
                    w381 = u32 0 ("分数")
                    n263 = property on="新形状触发源" class="Bool (strict)"("Val(Sgnl)"=TRUE ("值(信号)")) -> ()  [unwired: 2 in, 2 out]
                    n264 = local write "行数"(w381) -> ()
                    n265 = local write "分数"(w381) -> ()
                  }
                }
              }
            }
          }
        }
      }
    }
  }
  n266 = while {
    stop <- w383 stop-if-true
    # "计时器事件"
    n267 = local read "速度"() -> (w384:i32)
    n268 = event shown="[2] \"退出\": Value Change" {
      selector: _ -> [_ _ _]
      dyn-events: _ -> [_ _ _]
      timeout: w384 -> [_ _ _]
      tunnel: [FALSE FALSE TRUE] -> w383
      event Timeout {
        n269 = event-data() -> ()  [unwired: 1 in, 3 out]
        n270 = local read "落下状态"() -> (w386:bool)
        n271 = case shown="False" w386 {
          frame False {
            n272 = property on="下落触发源" class="Bool (strict)"("Val(Sgnl)"=TRUE ("值(信号)")) -> ()  [unwired: 2 in, 2 out]
          }
          frame True {
          }
        }
      }
      event "下落触发源", "开始/暂停", "初始化状态": Value Change {
        n273 = event-data() -> ()  [unwired: 1 in, 5 out]
      }
      event "退出": Value Change {
        n274 = event-data() -> ()  [unwired: 1 in, 4 out]
      }
    }
  }
  n275 = flat-sequence {
    frame #0 {
      w390 = u32 0 ("行数")
      w401 = 4 ("维数大小")
      # "初始化数据"
      n276 = Initialize Array(u32 0 ("元素"), w401, w401) -> (→"新形状数组" →"当前形状数组":u32[][])
      n277 = Initialize Array(u32 0 ("元素"), 18 ("维数大小"), 10 ("维数大小")) -> (→"主窗数组":u32[][])
      n278 = local write "开始/暂停"(FALSE ("运行状态")) -> ()
      "分数" <- w390
      "行数" <- w390
      "速度" <- 1000 ("速度")
      "落下状态" <- FALSE ("落下状态")
      "结束状态" <- FALSE ("结束状态")
      "Y" <- i8 -3 ("Y")
      "X" <- i8 4 ("X")
      "初始化状态" <- TRUE ("初始化状态")
      "键按下状态" <- FALSE ("键按下状态")
      "最高分数" <- w390
      "最多行数" <- w390
    }
    frame #1 {
      w422 = "游戏" ("section")
      w428 = "成绩" ("section")
      w408 = u32 0 ("default value")
      # "读取游戏状态"
      n279 = call <vilib>:"Application Directory.vi"() -> ("Application Directory"=w427:path)
      n280 = Build Path(base path=w427, name or relative path="俄罗斯方块.ini" ("名称或相对路径")) -> (appended path=w429:path)
      "配置文件路径" <- w429
      n281 = call <vilib>:"Open Config Data.vi"("configuration file path"=w429) -> ("error out"=w431:errorcluster, "refnum"=w436:T1)  [unwired: 8 in, 1 out]
      n282 = call-poly <vilib>:"Read Key.vi"("section"=w428, "error in (no error)"=w431, "default value"=w408, "key"="分数", "refnum"=w436) -> ("error out"=w432:errorcluster, "value"=w407:u32, "refnum out"=w434:T1)  [unwired: 3 in, 1 out]
      n283 = local write "最高分数"(w407) -> ()
      n284 = call-poly <vilib>:"Read Key.vi"("section"=w428, "error in (no error)"=w432, "default value"=w408, "key"="行数", "refnum"=w434) -> ("error out"=w423:errorcluster, "value"=w406:u32, "refnum out"=w424:T1)  [unwired: 3 in, 1 out]
      n285 = local write "最多行数"(w406) -> ()
      n286 = call-poly <vilib>:"Read Key.vi"("section"=w422, "error in (no error)"=w423, "default value"=TRUE ("value"), "key"="结束状态", "refnum"=w424) -> ("error out"=w420:errorcluster, "value"=w419:bool, "refnum out"=w421:T1)  [unwired: 3 in, 1 out]
      n287 = case shown="False" w419 {
        tunnel: w422 -> [w449 _]
        tunnel: w421 -> [w448 w541]
        tunnel: w420 -> [w447 w540]
        tunnel: [w440 w540] -> w414
        tunnel: [w439 w541] -> w413
        tunnel: "您是否要加载上次未结束的游戏进度吗？" ("消息") -> [w445 _]
        tunnel: "加载" ("T按钮名称（“确定”）") -> [w444 _]
        tunnel: "删除" ("Center Button Text (\"No\")") -> [w443 _]
        tunnel: "游戏进度加载对话框" ("Window Title (\"\")") -> [w442 _]
        frame False {
          n288 = property on="绘图触发源" class="Bool (strict)"("Val(Sgnl)"=TRUE ("值(信号)")) -> (error out=w437:errorcluster)  [unwired: 2 in, 1 out]
          n289 = call <vilib>:"Three Button Dialog.vi"("Window Title (\"\")"=w442, "Right Button Text (\"Cancel\")"="跳过" ("Center Button Text (\"No\")"), "Center Button Text (\"No\")"=w443, "Left Button Text (\"Yes\")"=w444, "message"=w445) -> ("Which Button?"=w446:T2)  [unwired: 6 in]
          n290 = case shown="\"Left Button\"" w446 {
            tunnel: w449 -> [w453 w531 _]
            tunnel: w448 -> [w474 w535 w538]
            tunnel: w447 -> [w473 w534 w537]
            tunnel: [w451 w532 w537] -> w440
            tunnel: [w452 w533 w538] -> w439
            tunnel: w437 -> [_ _ _]
            frame "Left Button" {
              w450 = u32 0 ("default value")
              n291 = property on="初始化状态" class="Bool (strict)"("Val(Sgnl)"=FALSE ("值(信号)")) -> ()  [unwired: 2 in, 2 out]
              n292 = call-poly <vilib>:"Read Key.vi"("section"=w453, "error in (no error)"=w473, "default value"=w450, "key"="分数", "refnum"=w474) -> ("error out"=w493:errorcluster, "value"=w463:u32, "refnum out"=w494:T1)  [unwired: 3 in, 1 out]
              n293 = local write "分数"(w463) -> ()
              n294 = call-poly <vilib>:"Read Key.vi"("section"=w453, "error in (no error)"=w493, "default value"=w450, "key"="行数", "refnum"=w494) -> ("error out"=w492:errorcluster, "value"=w464:u32, "refnum out"=w491:T1)  [unwired: 3 in, 1 out]
              n295 = local write "行数"(w464) -> ()
              n296 = call-poly <vilib>:"Read Key.vi"("section"=w453, "error in (no error)"=w492, "default value"=FALSE, "key"="开始/暂停", "refnum"=w491) -> ("error out"=w488:errorcluster, "value"=w462:bool, "refnum out"=w489:T1)  [unwired: 3 in, 1 out]
              n297 = local write "开始/暂停"(w462) -> ()
              n298 = call-poly <vilib>:"Read Key.vi"("section"=w453, "error in (no error)"=w488, "default value"=FALSE, "key"="落下状态", "refnum"=w489) -> ("error out"=w485:errorcluster, "value"=w460:bool, "refnum out"=w486:T1)  [unwired: 3 in, 1 out]
              n299 = local write "落下状态"(w460) -> ()
              n300 = call-poly <vilib>:"Read Key.vi"("section"=w453, "error in (no error)"=w485, "default value"=u32 1000, "key"="速度", "refnum"=w486) -> ("error out"=w483:errorcluster, "value"=w459:u32, "refnum out"=w482:T1)  [unwired: 3 in, 1 out]
              n301 = local write "速度"(w459) -> ()
              n302 = call-poly <vilib>:"Read Key.vi"("section"=w453, "error in (no error)"=w483, "default value"=4, "key"="X", "refnum"=w482) -> ("error out"=w480:errorcluster, "value"=w458:i32, "refnum out"=w478:T1)  [unwired: 3 in, 1 out]
              n303 = local write "X"(w458) -> ()
              n304 = call-poly <vilib>:"Read Key.vi"("section"=w453, "error in (no error)"=w480, "default value"=0, "key"="Y", "refnum"=w478) -> ("error out"=w475:errorcluster, "value"=w457:i32, "refnum out"=w476:T1)  [unwired: 3 in, 1 out]
              n305 = local write "Y"(w457) -> ()
              n306 = for {
                N: 3 -> [_]
                tunnel: w476 -> [w506]
                tunnel: w475 -> [w505]
                tunnel: [w504] -> w454
                tunnel: [w503] -> w455
                tunnel: w453 -> [w502]
                tunnel: [w497] -> w472 mode=indexing
                i -> [w501]
                n307 = Equal To 0?(x=w501) -> (x = 0?=w500:bool)
                n308 = case shown="False" w500 {
                  tunnel: [w507 18] -> w499
                  tunnel: [w507 10] -> w498
                  frame False {
                    w507 = 4
                  }
                  frame True {
                  }
                }
                n309 = for {
                  N: w499 -> [_]
                  tunnel: w498 -> [w518]
                  tunnel: w506 -> [w517]
                  tunnel: w501 -> [w515]
                  tunnel: w505 -> [w514]
                  tunnel: [w513] -> w504
                  tunnel: [w512] -> w503
                  tunnel: w502 -> [w511]
                  tunnel: [w510] -> w497 mode=indexing
                  i -> [w516]
                  n310 = for {
                    N: w518 -> [_]
                    tunnel: w517 -> [w529]
                    tunnel: w516 -> [w527]
                    tunnel: w515 -> [w526]
                    tunnel: w514 -> [w523]
                    tunnel: [w522] -> w513
                    tunnel: [w521] -> w512
                    tunnel: w511 -> [w520]
                    tunnel: [w519] -> w510 mode=indexing
                    i -> [w525]
                    n311 = Format Into String(format string="A%dY%02dX%d" ("格式字符串"), w526, w527, w525) -> (resulting string=w528:string)  [unwired: 2 in, 1 out]
                    n312 = call-poly <vilib>:"Read Key.vi"("section"=w520, "error in (no error)"=w523, "key"=w528, "refnum"=w529) -> ("error out"=w521:errorcluster, "value"=w519:u32, "refnum out"=w522:T1)  [unwired: 4 in, 1 out]
                  }
                }
              }
              n313 = call <vilib>:"Remove Section.vi"("section"=w453, "error in (no error)"=w455, "refnum"=w454) -> ("error out"=w451:errorcluster, "refnum out"=w452:T1)  [unwired: 6 in, 1 out]
              n314 = Index Array(array=w472) -> (element #1=w471:u32[][], element #2=w470:u32[][], element #3=w469:u32[][])  [unwired: 9 in]
              n315 = local write "当前形状数组"(w470) -> ()
              n316 = local write "新形状数组"(w469) -> ()
              n317 = local write "主窗数组"(w471) -> ()
            }
            frame "Center Button" {
              n318 = call <vilib>:"Remove Section.vi"("section"=w531, "error in (no error)"=w534, "refnum"=w535) -> ("error out"=w532:errorcluster, "refnum out"=w533:T1)  [unwired: 6 in, 1 out]
              n319 = property on="新形状触发源" class="Bool (strict)"("Val(Sgnl)"=TRUE ("值(信号)")) -> ()  [unwired: 2 in, 2 out]
            }
            frame "Right Button", Default {
              n320 = property on="新形状触发源" class="Bool (strict)"("Val(Sgnl)"=TRUE ("值(信号)")) -> ()  [unwired: 2 in, 2 out]
            }
          }
        }
        frame True {
          n321 = property on="新形状触发源" class="Bool (strict)"("Val(Sgnl)"=TRUE ("值(信号)")) -> ()  [unwired: 2 in, 2 out]
        }
      }
      n322 = call <vilib>:"Close Config Data.vi"("error in (no error)"=w414, "write file if changed (T)"=TRUE, "refnum"=w413) -> ("error out"=w418:errorcluster)  [unwired: 7 in, 1 out]
      n323 = call <vilib>:"Clear Errors.vi"("error in (no error)"=w418) -> ("error out"=w416:errorcluster)  [unwired: 5 in, 1 out]
      n324 = property on="绘图触发源" class="Bool (strict)"(error in=w416, "Val(Sgnl)"=TRUE ("值(信号)")) -> ()  [unwired: 1 in, 2 out]
    }
  }
